vi "Message decoding.vi"(8 "error in (no error)":errorcluster, 10 "Message":string, 11 "TCP Text Listener in":refnum<class "TCP Text Listener.lvclass">) -> (0 "error out":errorcluster, 2 "Message decoded":T1, 3 "TCP Text Listener out":refnum<class "TCP Text Listener.lvclass">)   [LabVIEW 2020, in "TALOS.lvlib" / "TCP Text Listener.lvlib" / "TCP Text Listener.lvclass"]
uses:
  TCP Text Listener.lvclass
  TCP Text Listener.lvclass/TCP Text Listener.ctl
  Support VIs/Global Constants.vi
  TALOS.lvlib
  TCP Writer/TCP Writer/TCP Message Internal Composition.ctl
  TCP Writer/TCP Writer/TCP Writer.lvclass
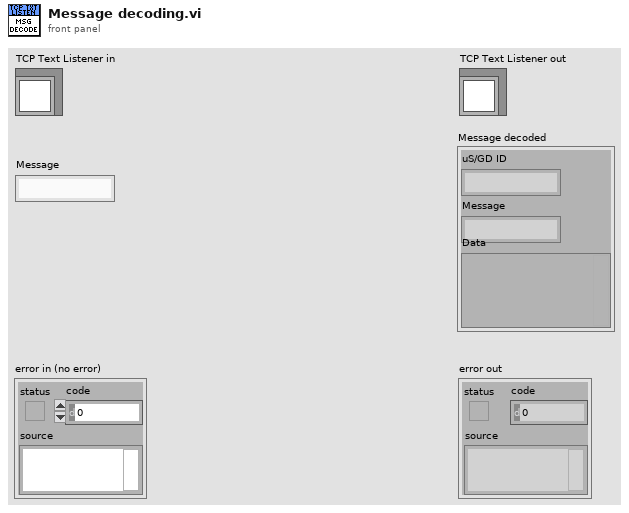
[diagram p1: front panel]
types:
  T1 = typedef "TALOS.lvlib/TCP Writer.lvlib/TCP Writer.lvclass/TCP Message Internal Composition.ctl" = cluster{"uS/GD ID":string, "Message":string, "Data":variant}
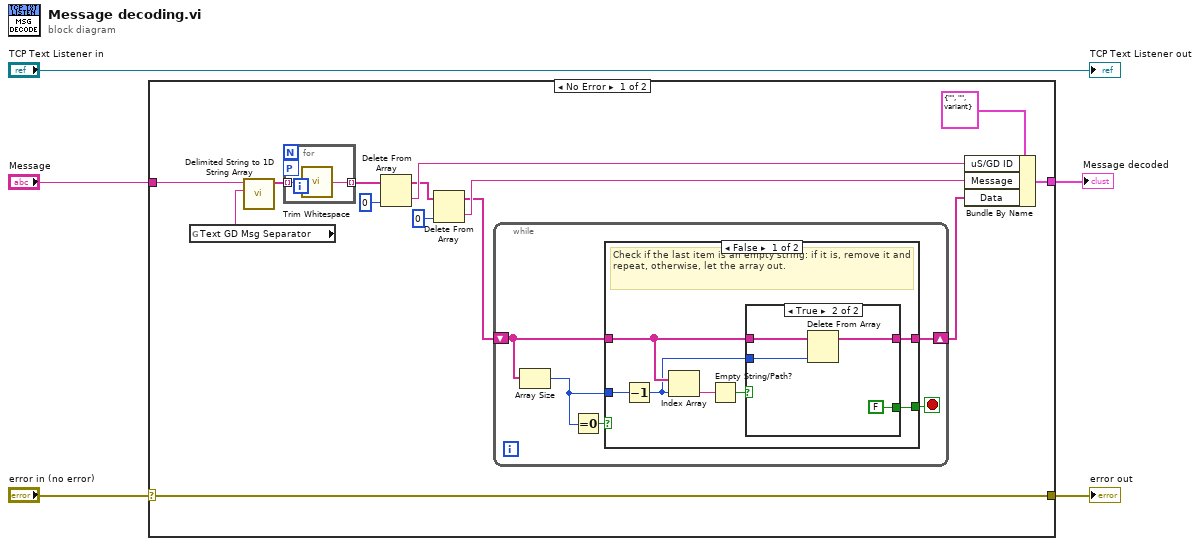
[diagram p0: block diagram]
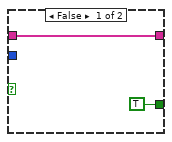
[diagram p2: hidden frame]
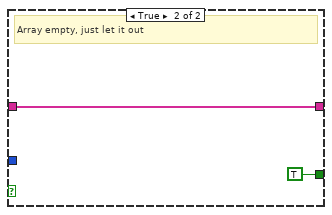
[diagram p3: hidden frame]
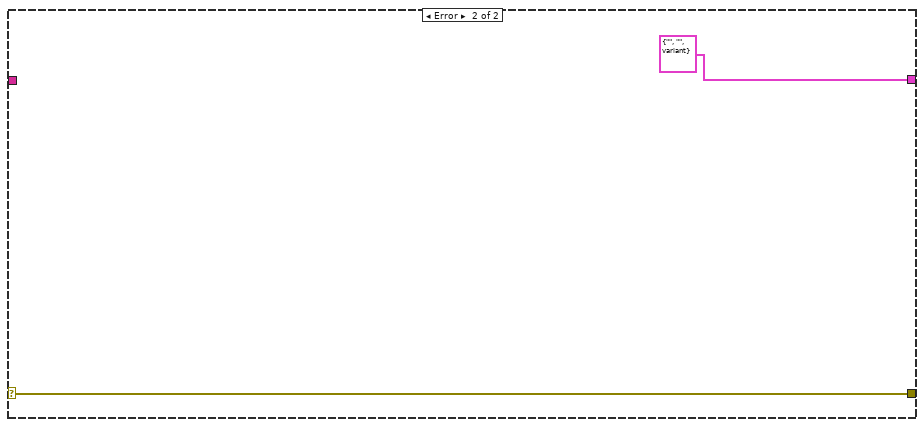
[diagram p4: hidden frame]
diagram:
  n1 = case shown="No Error" "error in (no error)" {
    selector: "error in (no error)" -> [w6 w42]
    tunnel: "Message" -> [w10 _]
    tunnel: [w7 T1 {"uS/GD ID"="", "Message"="", "Data"=variant} ("TCP Message Internal Composition")] -> w3
    tunnel: [w6 w42] -> w1
    frame No Error {
      n2 = global read "Global Constants.vi" "Text GD Msg Separator"() -> (w9:string)
      n3 = call <vilib>:"Delimited String to 1D String Array.vi"("delimiter"=w9, "delimited string"=w10) -> ("string array"=w19:string[])  [unwired: 9 in]
      n4 = for {
        tunnel: w19 -> [w41] mode=indexing
        tunnel: [w40] -> w18 mode=indexing
        workers-P: _ -> [_]
        n5 = call <vilib>:"Trim Whitespace.vi"("string"=w41) -> ("trimmed string"=w40:string)  [unwired: 1 in]
      }
      n6 = Delete From Array(array=w18, index=0) -> (deleted portion=w16:string, array with subset deleted=w15:string[])  [unwired: 1 in]
      n7 = Delete From Array(array=w15, index=0) -> (deleted portion=w13:string, array with subset deleted=w12:string[])  [unwired: 1 in]
      n8 = while {
        shift-right: [w21] -> w11
        shift-left: w12 -> [w22]
        stop <- w20 stop-if-true
        n9 = Array Size(array=w22) -> (size(s)=w24:i32)
        n10 = Equal To 0?(x=w24) -> (x = 0?=w23:bool)
        n11 = case shown="False" w23 {
          tunnel: w24 -> [w31 _]
          tunnel: w22 -> [w27 w39]
          tunnel: [w28 w39] -> w21
          tunnel: [w26 TRUE] -> w20
          frame False {
            # "Check if the last item is an empty string: if it is, remove it and repeat, otherwise, let the array out."
            n12 = Decrement(x=w31) -> (x-1=w25:i32)
            n13 = Index Array(array=w27, index=w25) -> (element=w30:string)
            n14 = Empty String/Path?(string/path=w30) -> (empty?=w29:bool)
            n15 = case shown="True" w29 {
              tunnel: [w33 w35] -> w28
              tunnel: w27 -> [w33 w37]
              tunnel: [TRUE FALSE] -> w26
              tunnel: w25 -> [_ w36]
              frame False {
              }
              frame True {
                n16 = Delete From Array(array=w37, index=w36) -> (array with subset deleted=w35:string[])  [unwired: 1 in, 1 out]
              }
            }
          }
          frame True {
            # "Array empty, just let it out"
          }
        }
      }
      n17 = Bundle By Name(cluster=T1 {"uS/GD ID"="", "Message"="", "Data"=variant} ("TCP Message Internal Composition"), "uS/GD ID"=w16, "Message"=w13, "Data"=w11) -> (w7:T1)
    }
    frame Error {
    }
  }
  "error out" <- w1
  "Message decoded" <- w3
  "TCP Text Listener out" <- "TCP Text Listener in"
